vi "Lire config EDWARDS.vi"(2 "error in (no error)":errorcluster caption="entrée d'erreur (pas d'erreur)", 3 "refnum":T2) -> (0 "error out":errorcluster, 1 "refnum out":T2)   [LabVIEW 2022 SP3]
uses:
  <vilib>/Utility/config.llb/Config Data RefNum.ctl
  Gestion grappe/TypeDef_Seuil Jauge Pression_CN.ctl
  <vilib>/Utility/config.llb/Read Key (String).vi
  <vilib>/Utility/config.llb/Read Key (Boolean).vi
  <vilib>/Utility/config.llb/Read Key (Double).vi
  Variables globales/Variable glob Edwards.vi
  <vilib>/Utility/config.llb/NI_LVConfig.lvlib
panel:
  out "Seuil Jauge":T1={"Descente en Pression"={"Min Mesure Piezo"=5.0, "Min Mesure Pirani"=0.0002}, "Montée en Pression"={"Max Mesure Pirani"=10.0, "Max Mesure Penning"=0.0004}} {"Montée en Pression"."Max Mesure Penning" format="%.2e"; "Montée en Pression"."Max Mesure Pirani" format="%.2e"; "Descente en Pression"."Min Mesure Pirani" format="%.2e"; "Descente en Pression"."Min Mesure Piezo" format="%.2e"}
  out "Grappes":string[][](array[string])
  out "Voies EDWARDS":u8[][](array[numeric])=[[1, 1], [1, 0]] max=6
  out "Noms jauges":string[][](array[string])
  out "Ports COM EDWARDS":refnum<visa-resource-name>[](array[refnum])
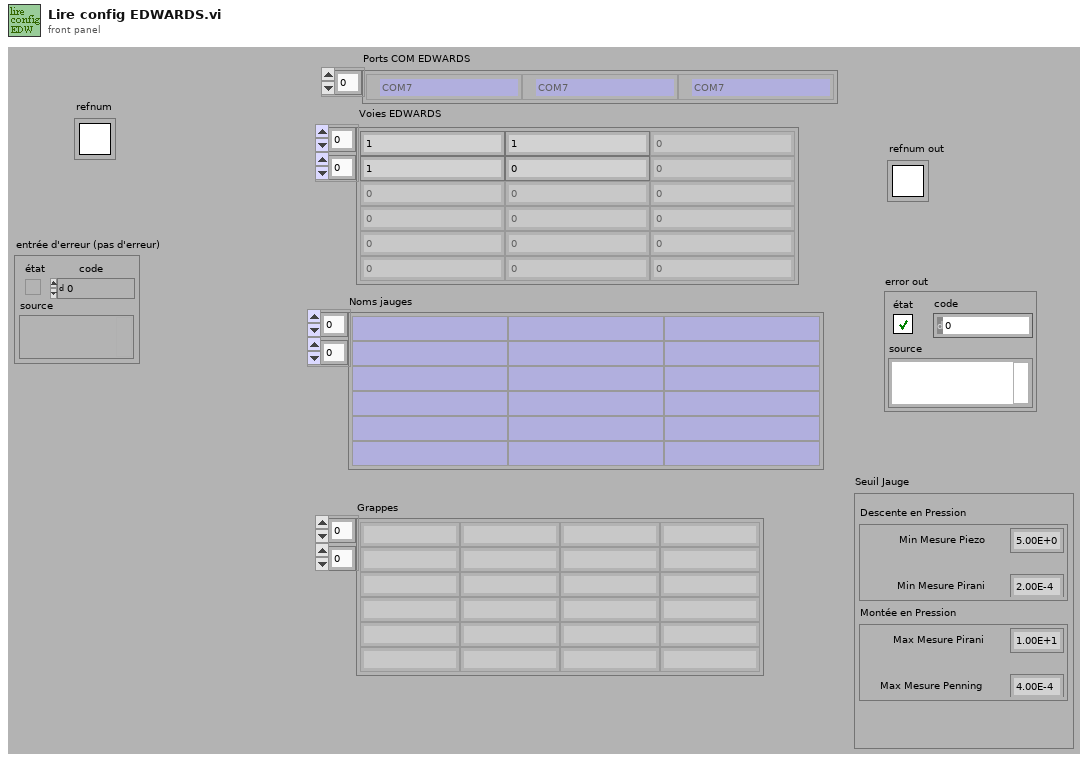
[diagram p1: front panel]
types:
  T1 = typedef "TypeDef_Seuil Jauge Pression_CN.ctl" = cluster{"Descente en Pression":cluster{"Min Mesure Piezo":dbl, "Min Mesure Pirani":dbl}, "Montée en Pression":cluster{"Max Mesure Pirani":dbl, "Max Mesure Penning":dbl}}
  T2 = typedef "NI_LVConfig.lvlib/Config Data RefNum.ctl" = refnum<k1>
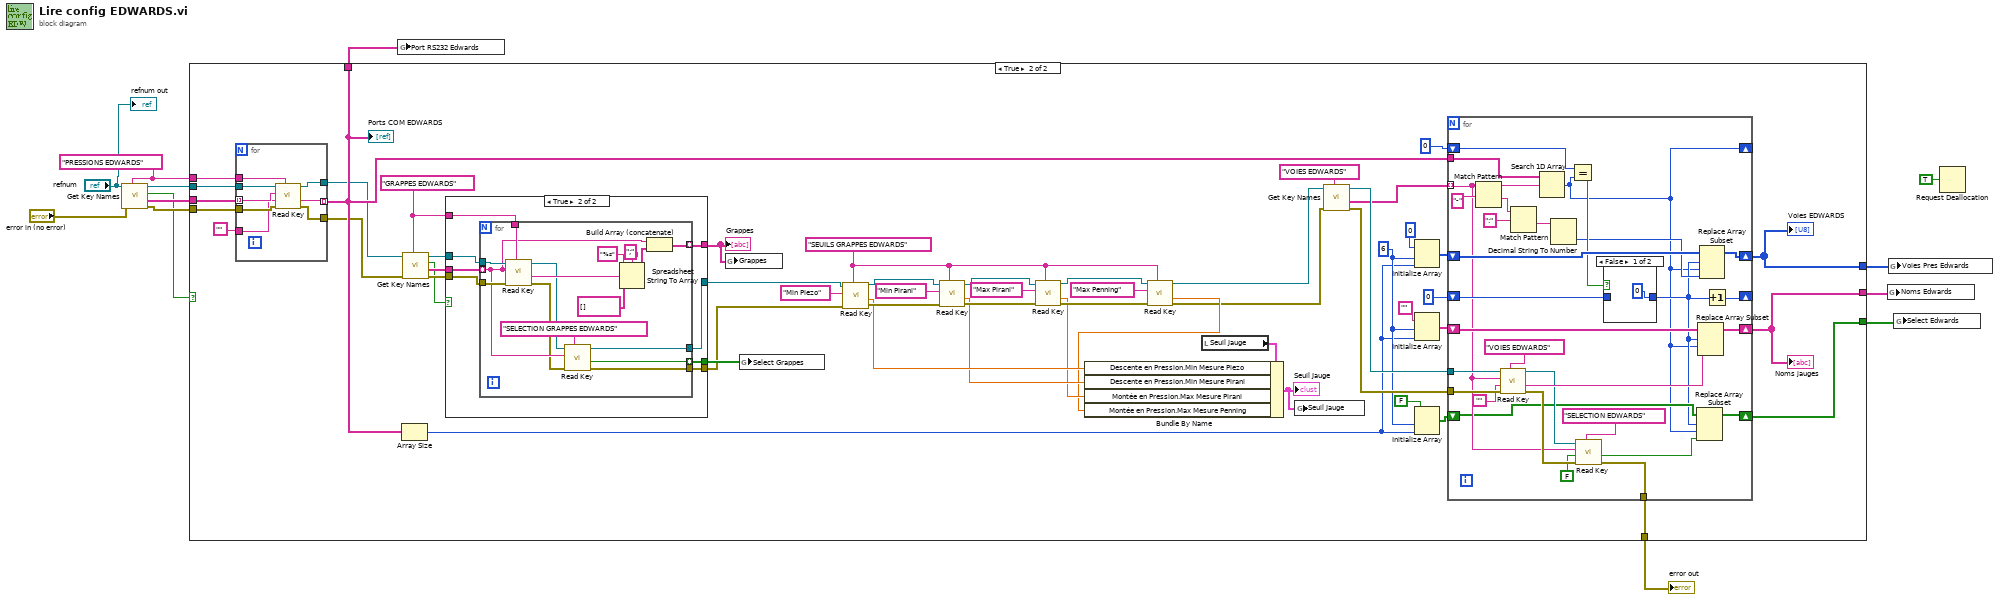
[diagram p0: block diagram]
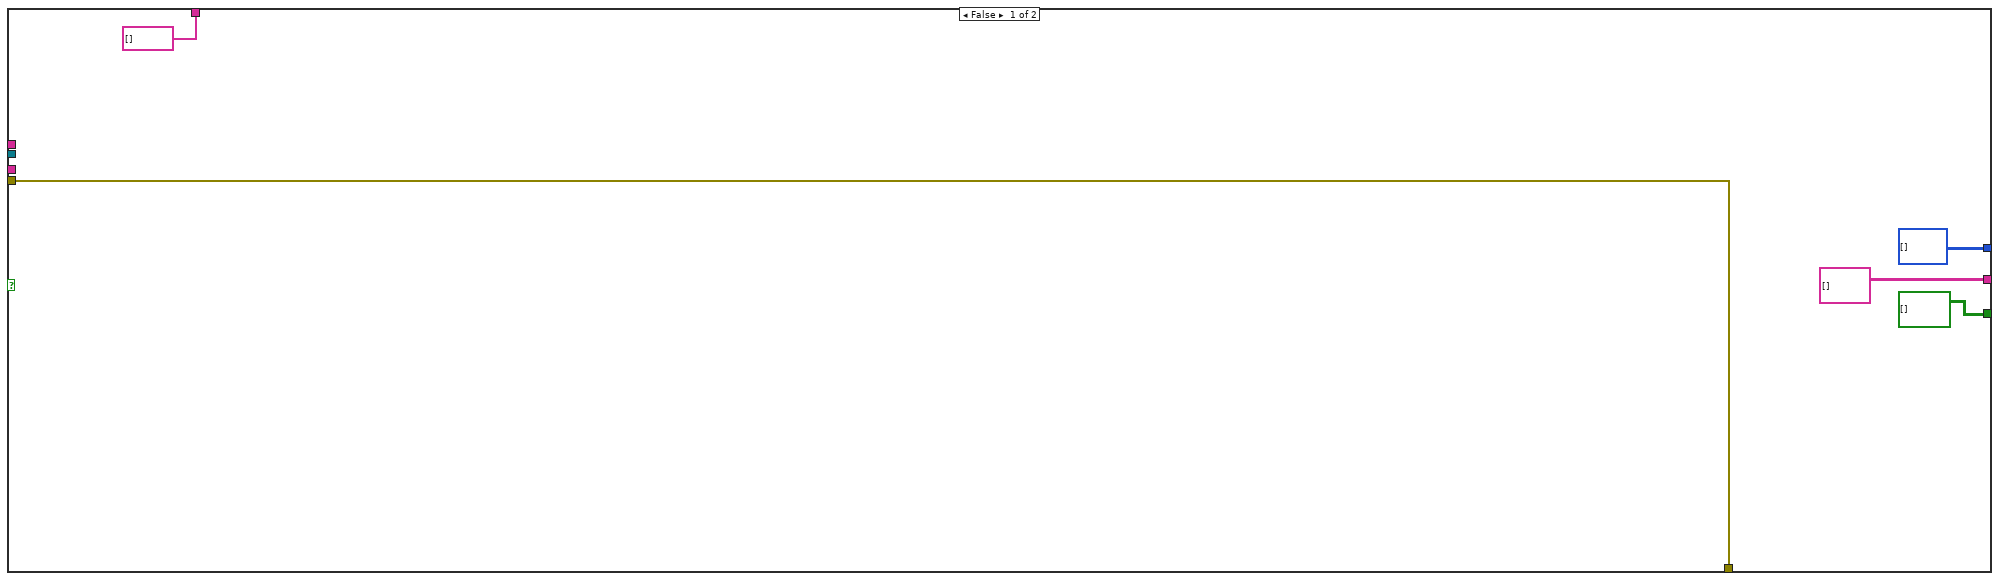
[diagram p2: hidden frame]
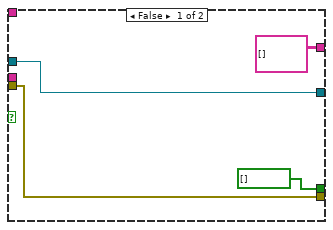
[diagram p3: hidden frame]
diagram:
  w10 = "PRESSIONS EDWARDS" ("section")
  n1 = call <vilib>:"Get Key Names.vi"("section"=w10, "error in (no error)"="error in (no error)", "refnum"="refnum") -> ("error out"=w11:errorcluster, "key names"=w13:string[], "section exists?"=w6:bool, "refnum out"=w12:T2)  [unwired: 5 in]
  n2 = case shown="True" w6 {
    tunnel: w13 -> [_ w72]
    tunnel: w12 -> [_ w71]
    tunnel: w11 -> [w17 w70]
    tunnel: w10 -> [_ w69]
    tunnel: [w17 w68] -> w9
    tunnel: [bool[][] [] w67] -> w3
    tunnel: [string[] [] w66] -> w7
    tunnel: [i32[][] [] w65] -> w5
    tunnel: [string[][] [] w64] -> w4
    frame False {
    }
    frame True {
      w21 = "SEUILS GRAPPES EDWARDS" ("section")
      w48 = "GRAPPES EDWARDS" ("section")
      w51 = 6 ("taille de la dimension")
      n3 = for {
        tunnel: w72 -> [w138] mode=indexing
        tunnel: w71 -> [w141]
        tunnel: w70 -> [w140]
        tunnel: w69 -> [w139]
        tunnel: "" -> [w137]
        tunnel: [w136] -> w66 mode=indexing
        tunnel: [w135] -> w45
        tunnel: [w134] -> w44
        n4 = call-poly <vilib>:"Read Key.vi"("section"=w139, "error in (no error)"=w140, "default value"=w137, "key"=w138, "refnum"=w141) -> ("error out"=w134:errorcluster, "value"=w136:string, "refnum out"=w135:T2)  [unwired: 3 in, 1 out]
      }
      "Ports COM EDWARDS" <- w66
      n5 = Array Size(array=w66) -> (size(s)=w50:i32)
      n6 = call <vilib>:"Get Key Names.vi"("section"=w48, "error in (no error)"=w44, "refnum"=w45) -> ("error out"=w42:errorcluster, "key names"=w47:string[], "section exists?"=w19:bool, "refnum out"=w43:T2)  [unwired: 5 in]
      n7 = case shown="True" w19 {
        tunnel: w48 -> [_ w84]
        tunnel: w47 -> [_ w83]
        tunnel: [string[][] [] w82] -> w46
        tunnel: w43 -> [w76 w81]
        tunnel: w42 -> [w75 w80]
        tunnel: [bool[] [] w79] -> w41
        tunnel: [w76 w78] -> w40
        tunnel: [w75 w77] -> w39
        frame False {
        }
        frame True {
          n8 = for {
            tunnel: w84 -> [w100]
            tunnel: w83 -> [w91] mode=indexing
            tunnel: [w94] -> w82 mode=indexing
            tunnel: w81 -> [w93]
            tunnel: w80 -> [w92]
            tunnel: [w89] -> w79 mode=indexing
            tunnel: [w86] -> w78
            tunnel: [w85] -> w77
            n9 = call-poly <vilib>:"Read Key.vi"("section"=w100, "error in (no error)"=w92, "key"=w91, "refnum"=w93) -> ("error out"=w87:errorcluster, "value"=w99:string, "refnum out"=w88:T2)  [unwired: 4 in, 1 out]
            n10 = call-poly <vilib>:"Read Key.vi"("section"="SELECTION GRAPPES EDWARDS", "error in (no error)"=w87, "key"=w91, "refnum"=w88) -> ("error out"=w85:errorcluster, "value"=w89:bool, "refnum out"=w86:T2)  [unwired: 4 in, 1 out]
            n11 = Spreadsheet String To Array(delimiter (Tab)=";" ("séparateur (Tabulation)"), format string="%s" ("chaîne de format"), spreadsheet string=w99, array type (2D Dbl)=string[] [] ("type de tableau (2D de dbl)")) -> (array=w95:string[])
            n12 = Build Array (concatenate)(w91, w95) -> (w94:string[])
          }
        }
      }
      "Grappes" <- w46
      n13 = global write "Variable glob Edwards.vi" "Grappes"(w46) -> ()
      n14 = global write "Variable glob Edwards.vi" "Select Grappes"(w41) -> ()
      n15 = call-poly <vilib>:"Read Key.vi"("section"=w21, "error in (no error)"=w39, "key"="Min Piezo", "refnum"=w40) -> ("error out"=w35:errorcluster, "value"=w27:dbl, "refnum out"=w36:T2)  [unwired: 4 in, 1 out]
      n16 = call-poly <vilib>:"Read Key.vi"("section"=w21, "error in (no error)"=w35, "key"="Min Pirani", "refnum"=w36) -> ("error out"=w32:errorcluster, "value"=w26:dbl, "refnum out"=w33:T2)  [unwired: 4 in, 1 out]
      n17 = call-poly <vilib>:"Read Key.vi"("section"=w21, "error in (no error)"=w32, "key"="Max Pirani", "refnum"=w33) -> ("error out"=w29:errorcluster, "value"=w25:dbl, "refnum out"=w30:T2)  [unwired: 4 in, 1 out]
      n18 = call-poly <vilib>:"Read Key.vi"("section"=w21, "error in (no error)"=w29, "key"="Max Penning", "refnum"=w30) -> ("error out"=w22:errorcluster, "value"=w24:dbl, "refnum out"=w23:T2)  [unwired: 4 in, 1 out]
      n19 = local read "Seuil Jauge"() -> (w28:T1)
      n20 = Bundle By Name(cluster=w28, "Descente en Pression.Min Mesure Piezo"=w27, "Descente en Pression.Min Mesure Pirani"=w26, "Montée en Pression.Max Mesure Pirani"=w25, "Montée en Pression.Max Mesure Penning"=w24) -> (w20:T1)
      "Seuil Jauge" <- w20
      n21 = global write "Variable glob Edwards.vi" "Seuil Jauge"(w20) -> ()
      n22 = call <vilib>:"Get Key Names.vi"("section"="VOIES EDWARDS", "error in (no error)"=w22, "refnum"=w23) -> ("error out"=w60:errorcluster, "key names"=w53:string[], "refnum out"=w59:T2)  [unwired: 5 in, 1 out]
      n23 = Initialize Array(0 ("taille de la dimension"), w51, w50) -> (w57:i32[][])
      n24 = Initialize Array("", w51, w50) -> (w61:string[][])
      n25 = Initialize Array(FALSE, w51, w50) -> (w49:bool[][])
      n26 = for {
        tunnel: w53 -> [w107] mode=indexing
        tunnel: w66 -> [w130]
        shift-right: [w102] -> _
        shift-left: 0 -> [w125]
        shift-right: [w121] -> w65
        shift-left: w57 -> [w122]
        shift-right: [w123] -> _
        shift-left: 0 -> [w124]
        tunnel: w59 -> [w119]
        tunnel: w60 -> [w118]
        shift-right: [w112] -> w64
        shift-left: w61 -> [w115]
        tunnel: [w109] -> w68
        shift-right: [w104] -> w67
        shift-left: w49 -> [w105]
        n27 = Match Pattern(string=w107, regular expression="-" ("expression régulière")) -> (before substring=w129:string, after substring=w128:string)  [unwired: 1 in, 2 out]
        n28 = call-poly <vilib>:"Read Key.vi"("section"="VOIES EDWARDS", "error in (no error)"=w118, "default value"="", "key"=w107, "refnum"=w119) -> ("error out"=w110:errorcluster, "value"=w113:string, "refnum out"=w111:T2)  [unwired: 3 in, 1 out]
        n29 = Match Pattern(string=w128, regular expression=":" ("expression régulière")) -> (after substring=w126:string)  [unwired: 1 in, 3 out]
        n30 = Search 1D Array(1D array=w130, element=w129) -> (index of element=w102:i32)  [unwired: 1 in]
        n31 = Decimal String To Number(string=w126) -> (number=w114:i32)  [unwired: 2 in, 1 out]
        n32 = Equal?(x=w125, y=w102) -> (x = y?=w120:bool)
        n33 = call-poly <vilib>:"Read Key.vi"("section"="SELECTION EDWARDS", "error in (no error)"=w110, "default value"=FALSE, "key"=w107, "refnum"=w111) -> ("error out"=w109:errorcluster, "value"=w101:bool)  [unwired: 3 in, 2 out]
        n34 = case shown="False" w120 {
          tunnel: w124 -> [_ w133]
          tunnel: [0 w133] -> w103
          frame False {
          }
          frame True {
          }
        }
        n35 = Replace Array Subset(array=w105, new element=w101, index (row)=w103, index (col)=w102) -> (w104:bool[][])
        n36 = Replace Array Subset(array=w115, new element=w113, index (row)=w103, index (col)=w102) -> (w112:string[][])
        n37 = Replace Array Subset(array=w122, new element=w114, index (row)=w103, index (col)=w102) -> (w121:i32[][])
        n38 = Increment(x=w103) -> (x+1=w123:i32)
      }
      "Voies EDWARDS" <- w65
      "Noms jauges" <- w64
    }
  }
  "error out" <- w9
  n39 = global write "Variable glob Edwards.vi" "Port RS232 Edwards"(w7) -> ()
  n40 = global write "Variable glob Edwards.vi" "Noms Edwards"(w4) -> ()
  n41 = global write "Variable glob Edwards.vi" "Voies Pres Edwards"(w5) -> ()
  n42 = global write "Variable glob Edwards.vi" "Select Edwards"(w3) -> ()
  n43 = Request Deallocation(TRUE ("flag")) -> ()
  "refnum out" <- "refnum"
